vi "Get Board.vi"(8 "error in (no error)":errorcluster) -> (0 "error out":errorcluster, 1 "Model Number":i32, 2 "Memory":string, 3 "Model":string)   [LabVIEW 2020, in "wiringPi.lvlib"]
doc: "<b>_______________________________________________________________</b>\n** Author: Juan José Villacorta\n** LabVIEW wrapper for C library <b> wiringPi </b>,\n** https://github.com/WiringPi/WiringPi\n<b>_______________________________________________________________</b>\n\n*\n * piBoardId:\n * Return the real details of the board we have.\n *\n * This is undocumented and really only intended for the GPIO command.\n * Use at your own risk!\n *\n*/\n\n/*\n * wiringPiSetupGpio:\n * Must be called once at the start of your program execution.\n *\n * GPIO setup: Initialises the system into GPIO Pin mode and uses the\n * memory mapped hardware directly.\n *********************************************************************************\n */"
uses:
  wiringPi.lvlib
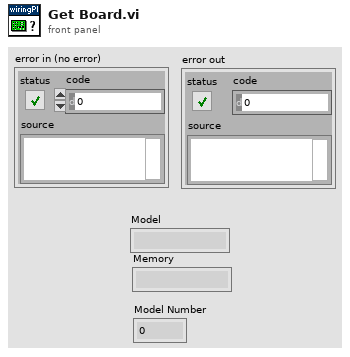
[diagram p1: front panel]
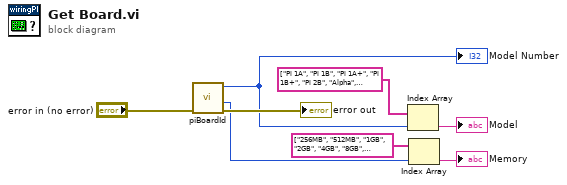
[diagram p0: block diagram]
diagram:
  n1 = call "piBoardId.vi"("error in (no error)"="error in (no error)") -> ("error out"=→"error out":errorcluster, "mem"=w1:i32, "Model Number"=w2:i32)  [unwired: 5 in, 3 out]
  "Model Number" <- w2
  n2 = Index Array(array=string[] ["Pi 1A", "Pi 1B", "Pi 1A+", "Pi 1B+", "Pi 2B", "Alpha", "CM1", "-", "Pi  3B", "Pi Zero", "CM3", "-", "Pi Zero W", "Pi 3B+", "Pi 3A+", "-", "CM3+", "Pi 4B", "Zero 2W", "400", "CM4", "CM4S", "-", "Pi 5", "CM5", "500", "CM5 Lite"], index=w2) -> (element=→"Model":string)
  n3 = Index Array(array=string[] ["256MB", "512MB", "1GB", "2GB", "4GB", "8GB", "16GB"], index=w1) -> (element=→"Memory":string)
